vi "String To Number(U64).vi"(5 "String":string) -> (0 "Numeric(U64)":u64)   [LabVIEW 2017]
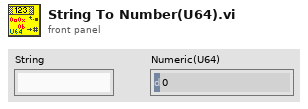
[diagram p1: front panel]
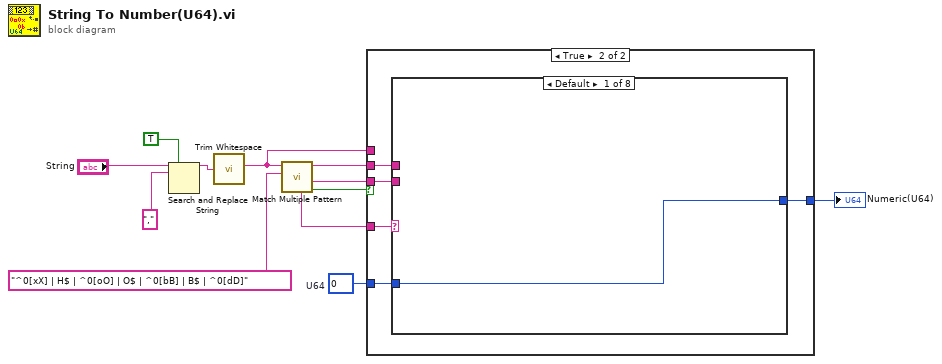
[diagram p0: block diagram]
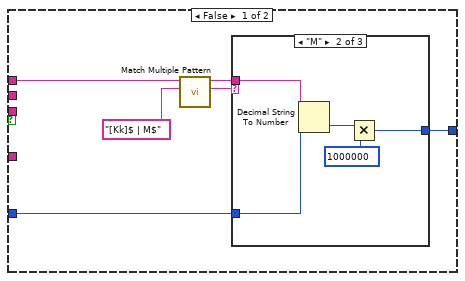
[diagram p2: hidden frame]
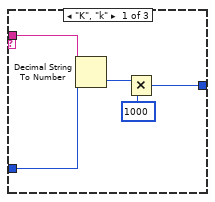
[diagram p3: hidden frame]
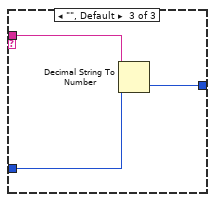
[diagram p4: hidden frame]
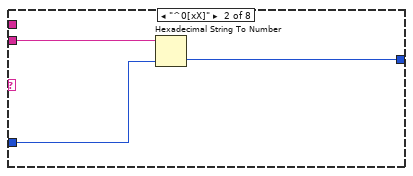
[diagram p5: hidden frame]
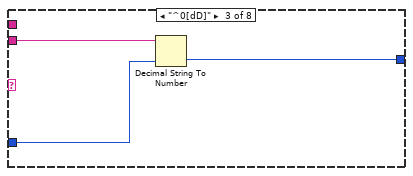
[diagram p6: hidden frame]
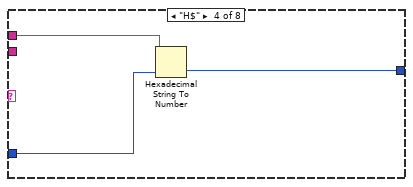
[diagram p7: hidden frame]
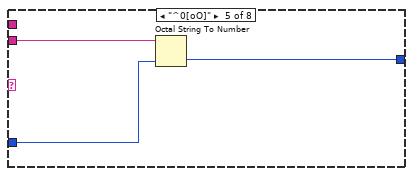
[diagram p8: hidden frame]
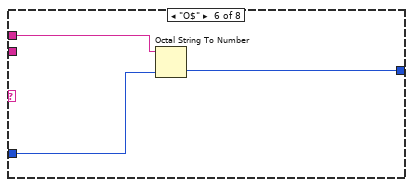
[diagram p9: hidden frame]
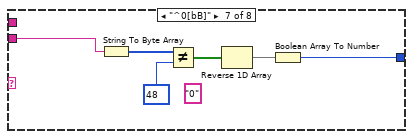
[diagram p10: hidden frame]
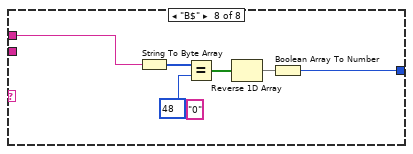
[diagram p11: hidden frame]
diagram:
  w1 = u64 0  # U64
  n1 = Search and Replace String(replace all?=TRUE ("replace all? (F)"), input string="String", search string=",") -> (result string=w9:string)  [unwired: 5 in, 3 out]
  n2 = call <vilib>:"Trim Whitespace.vi"("string"=w9) -> ("trimmed string"=w2:string)  [unwired: 1 in]
  n3 = call "Match Multiple Pattern.vi"("regular expression"="^0[xX] | H$ | ^0[oO] | O$ | ^0[bB] | B$ | ^0[dD]", "string"=w2) -> ("Found?"=w7:bool, "after substring"=w5:string, "before substring"=w4:string, "pattern matched"=w6:string)  [unwired: 5 in, 1 out]
  n4 = case shown="True" w7 {
    tunnel: w6 -> [_ w36]
    tunnel: w5 -> [_ w35]
    tunnel: w4 -> [_ w34]
    tunnel: [w18 w33] -> w3
    tunnel: w2 -> [w16 _]
    tunnel: w1 -> [w17 w32]
    frame False {
      n5 = call "Match Multiple Pattern.vi"("regular expression"="[Kk]$ | M$", "string"=w16) -> ("match substring"=w14:string, "before substring"=w13:string)  [unwired: 5 in, 3 out]
      n6 = case shown="\"M\"" w14 {
        tunnel: [w19 w24 w31] -> w18
        tunnel: w17 -> [w22 w27 w30]
        tunnel: w13 -> [w23 w28 w29]
        frame "K", "k" {
          n7 = Decimal String To Number(string=w23, default (0L)=w22) -> (number=w21:u64)  [unwired: 1 in, 1 out]
          n8 = Multiply(x=w21, y=u64 1000) -> (x*y=w19:u64)
        }
        frame "M" {
          n9 = Decimal String To Number(string=w28, default (0L)=w27) -> (number=w26:u64)  [unwired: 1 in, 1 out]
          n10 = Multiply(x=w26, y=u64 1000000) -> (x*y=w24:u64)
        }
        frame "", Default {
          n11 = Decimal String To Number(string=w29, default (0L)=w30) -> (number=w31:u64)  [unwired: 1 in, 1 out]
        }
      }
    }
    frame True {
      n12 = case shown="Default" w36 {
        tunnel: w35 -> [_ w40 w43 _ w49 _ w57 _]
        tunnel: w34 -> [_ _ _ w45 _ w51 _ w61]
        tunnel: [w37 w39 w42 w46 w48 w52 w58 w64] -> w33
        tunnel: w32 -> [w37 w38 w41 w44 w47 w50 _ _]
        frame Default {
        }
        frame "^0[xX]" {
          n13 = Hexadecimal String To Number(string=w40, default (0uL)=w38) -> (number=w39:u64)  [unwired: 1 in, 1 out]
        }
        frame "^0[dD]" {
          n14 = Decimal String To Number(string=w43, default (0L)=w41) -> (number=w42:u64)  [unwired: 1 in, 1 out]
        }
        frame "H$" {
          n15 = Hexadecimal String To Number(string=w45, default (0uL)=w44) -> (number=w46:u64)  [unwired: 1 in, 1 out]
        }
        frame "^0[oO]" {
          n16 = Octal String To Number(2:w47, 4:w49) -> (0:w48:u64)  [unwired: 1 in, 1 out]
        }
        frame "O$" {
          n17 = Octal String To Number(2:w50, 4:w51) -> (0:w52:u64)  [unwired: 1 in, 1 out]
        }
        frame "^0[bB]" {
          (unwired) "0" ("search string")
          n18 = String To Byte Array(string=w57) -> (unsigned byte array=w56:u8[])
          n19 = Not Equal?(x=w56, y=u8 48) -> (x != y?=w54:bool[])
          n20 = Reverse 1D Array(array=w54) -> (reversed array=w53:bool[])
          n21 = Boolean Array To Number(Boolean array=w53) -> (number=w58:u64)
        }
        frame "B$" {
          (unwired) "0" ("search string")
          n22 = String To Byte Array(string=w61) -> (unsigned byte array=w63:u8[])
          n23 = Equal?(x=w63, y=u8 48) -> (x = y?=w62:bool[])
          n24 = Reverse 1D Array(array=w62) -> (reversed array=w60:bool[])
          n25 = Boolean Array To Number(Boolean array=w60) -> (number=w64:u64)
        }
      }
    }
  }
  "Numeric(U64)" <- w3
